vi "Pre Launch Init.vi"(11 "Input Operator in":refnum<class "ControlPanel.lvclass"> caption="操作者输入") -> (0 "error out":errorcluster caption="错误输出", 3 "Input Operator out":refnum<class "ControlPanel.lvclass"> caption="操作者输出")   [LabVIEW 2014, in "ControlPanel.lvlib" / "ControlPanel.lvclass"]
doc: "(<B>Filename</B>: Actor Framework.lvlib:Actor.lvclass:Pre Launch Init.vi)\n\nDefines behavior that occurs after the Launch Nested Actor method is invoked but before the actor's Actor Core method begins running.\n\nBy default, this method does nothing. A descendant class may override it to define behavior."
uses:
  ControlPanel.lvclass
  ctl/P3AT_Current.ctl
  ControlPanel.lvclass/ControlPanel.ctl
  Global_var/Global_var.vi
  <vilib>/Utility/xml.llb/Read From XML File(array).vi
  <vilib>/Utility/xml.llb/Read From XML File(string).vi
  Wrapper_lib/zsActor/ActorWrapper.lvclass
panel:
  out "XML Elements":string caption="XML元素"
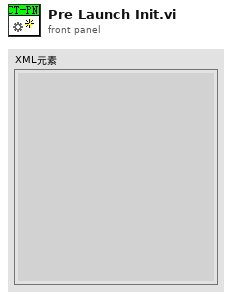
[diagram p1: front panel]
types:
  T1 = typedef "P3AT_Current.ctl" = cluster{"max_vel":dbl, "max_rot":dbl, "now_pose_X":dbl, "now_pose_Y":dbl, "now_pose_Rot_deg":dbl, "Control_Mode":enum32{"Joy", "Map", "Voice", "Input", "Undefined"}}
  T2 = enum16{"OpenSlaveActor", "Idle", "StopSlaveActor"}
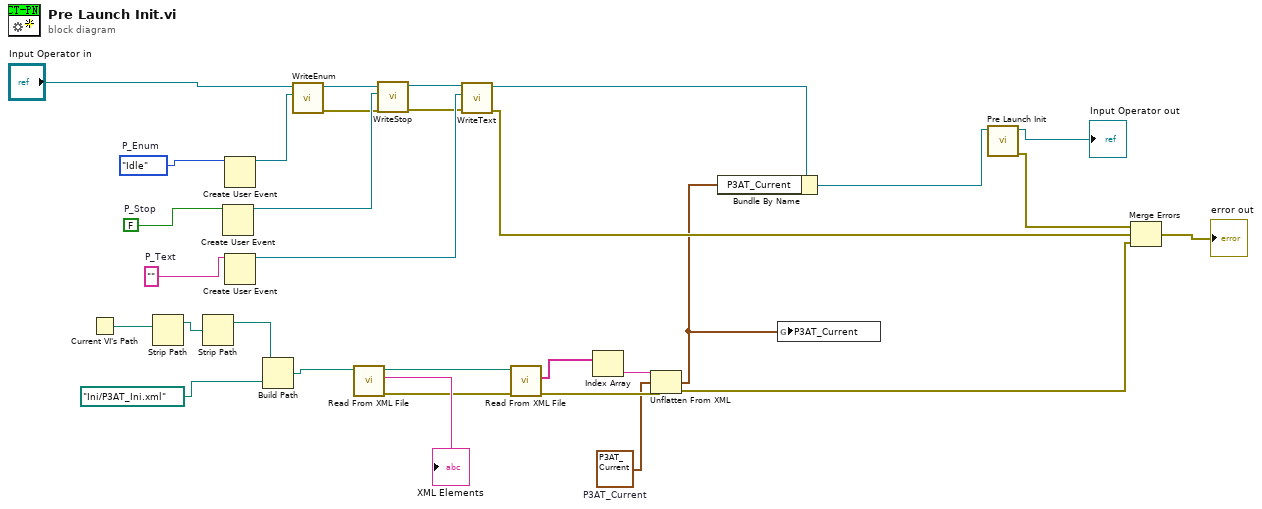
[diagram p0: block diagram]
diagram:
  w1 = T1 {"max_vel"=0.49056603773584906, "max_rot"=0.5094339622641509, "now_pose_X"=0.0, "now_pose_Y"=0.0, "now_pose_Rot_deg"=0.0, "Control_Mode"=enum."Joy"}  # P3AT_Current
  w12 = ""  # P_Text
  w11 = FALSE  # P_Stop
  w10 = T2."Idle"  # P_Enum
  n1 = Current VI's Path() -> (path=w20:path)
  n2 = Strip Path(path=w20) -> (stripped path=w21:path)  [unwired: 1 out]
  n3 = Strip Path(path=w21) -> (stripped path=w22:path)  [unwired: 1 out]
  n4 = Create User Event(user event datatype=w11) -> (user event=w8:refnum<user-event>)  [unwired: 1 in, 1 out]
  n5 = Create User Event(user event datatype=w10) -> (user event=w9:refnum<user-event>)  [unwired: 1 in, 1 out]
  n6 = Create User Event(user event datatype=w12) -> (user event=w7:refnum<user-event>)  [unwired: 1 in, 1 out]
  n7 = Build Path(base path=w22, name or relative path=path "Ini/P3AT_Ini.xml" ("拆分的路径")) -> (appended path=w19:path)
  n8 = call-dynamic "WriteEnum.vi"("Enum"=w9, "zsActor输入"="Input Operator in") -> ("error out"=w6:errorcluster, "zsActor输出"=w15:refnum<class "ControlPanel.lvclass">)  [unwired: 8 in]
  n9 = call-poly <vilib>:"Read From XML File.vi"("XML File Path"=w19) -> ("error out"=w18:errorcluster, "XML Elements"=→"XML Elements":string, "XML File Path(duplicate)"=w27:path)  [unwired: 8 in]
  n10 = call-dynamic "WriteStop.vi"("error in (no error)"=w6, "Stop"=w8, "zsActor输入"=w15) -> ("error out"=w5:errorcluster, "zsActor输出"=w14:refnum<class "ControlPanel.lvclass">)  [unwired: 7 in]
  n11 = call-dynamic "WriteText.vi"("error in (no error)"=w5, "Text"=w7, "zsActor输入"=w14) -> ("error out"=w4:errorcluster, "zsActor输出"=w13:refnum<class "ControlPanel.lvclass">)  [unwired: 7 in]
  n12 = call-poly <vilib>:"Read From XML File.vi"("error in (no error)"=w18, "XML File Path"=w27) -> ("error out"=w17:errorcluster, "XML Elements"=w25:string[])  [unwired: 7 in, 1 out]
  n13 = Index Array(array=w25) -> (element=w24:string)  [unwired: 1 in]
  n14 = Unflatten From XML(xml string=w24, type=w1, error in (no error)=w17) -> (value=w2:T1, error out=w3:errorcluster)
  n15 = Bundle By Name(cluster=w13, "P3AT_Current"=w2) -> (w30:refnum<class "ControlPanel.lvclass">)
  n16 = global write "Global_var.vi" "P3AT_Current"(w2) -> ()
  n17 = call-parent "Pre Launch Init.vi"("Actor in"=w30) -> ("error out"=w29:errorcluster, "Actor out"=→"Input Operator out":refnum<class "ControlPanel.lvclass">)  [unwired: 9 in]
  n18 = Merge Errors(w29, w4, w3) -> (→"error out":errorcluster)
